vi "Add Fixture Files.vi"(8 "error in (no error)":errorcluster, 11 "server id":i32) -> (0 "error out":errorcluster, 3 "server id out":i32)   [LabVIEW 2020, in "MCP Server tests.lvlib"]
doc: "Test helper. Registers the two fixture files that lie beside this VI as MCP resources: fixture_utf8.txt (UTF-8 text with non-ASCII characters and Windows line endings) and fixture_binary.png (a binary file)."
uses:
  MCP Server tests.lvlib
  src/MCP Server/MCP Server.lvlib
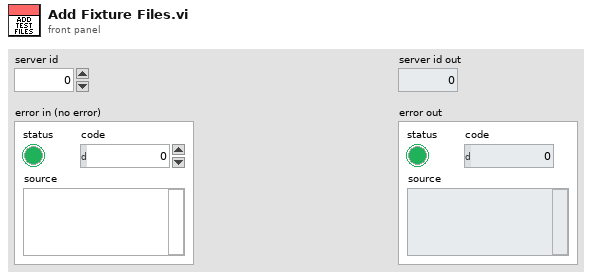
[diagram p1: front panel]
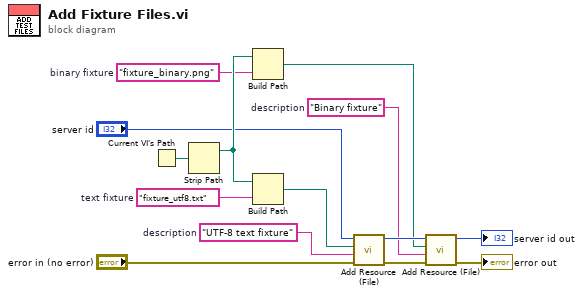
[diagram p0: block diagram]
diagram:
  w4 = "Binary fixture"  # description
  w8 = "UTF-8 text fixture"  # description
  w11 = "fixture_binary.png"  # binary fixture
  w13 = "fixture_utf8.txt"  # text fixture
  n1 = Current VI's Path() -> (path=w14:path)
  n2 = Strip Path(path=w14) -> (stripped path=w12:path)  [unwired: 1 out]
  n3 = Build Path(base path=w12, name or relative path=w11) -> (appended path=w5:path)
  n4 = Build Path(base path=w12, name or relative path=w13) -> (appended path=w9:path)
  n5 = call "Add Resource (File).vi"("error in (no error)"="error in (no error)", "description"=w8, "file path"=w9, "server id"="server id") -> ("error out"=w3:errorcluster, "server id out"=w6:i32)  [unwired: 6 in]
  n6 = call "Add Resource (File).vi"("error in (no error)"=w3, "description"=w4, "file path"=w5, "server id"=w6) -> ("error out"=→"error out":errorcluster, "server id out"=→"server id out":i32)  [unwired: 6 in]
